vi "Get Mode.vi"(8 "error in":errorcluster, 11 "Element in":refnum<class "Element.lvclass">) -> (0 "error out":errorcluster, 2 "Parameter Mode":T1, 3 "Element out":refnum<class "Element.lvclass">)   [LabVIEW 2026, in "Element.lvclass"]
doc: "Get Mode."
uses:
  Element.lvclass
  Type Definitions/Parameter Mode--enum.ctl
  Element.lvclass/Element.ctl
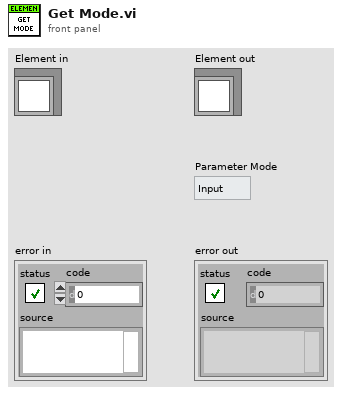
[diagram p1: front panel]
types:
  T1 = typedef "Parameter Mode--enum.ctl" = enum16{"Input", "Output"}
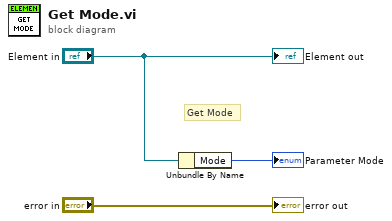
[diagram p0: block diagram]
diagram:
  # "Get Mode"
  n1 = Unbundle By Name("Element in") -> ("Mode"=→"Parameter Mode":T1)
  "error out" <- "error in"
  "Element out" <- "Element in"
